vi "VIH Dialog - VI Terminals - Term Symbols.vi"(6 "cmd (nop)":T2(ring), 8 "error in":errorcluster, 11 "Ctl Refnum":refnum<vi>) -> (0 "error out":errorcluster, 1 "Symbols":T1[](array[typedef]), 2 "Symbol Index":i32, 3 "dup Ctl Refnum":refnum<vi>)   [LabVIEW 2014]
doc: "::: VI Helpeks :::\nCopyright (c) 2000-2026 Konstantin Shifershteyn. All rights reserved."
uses:
  <vilib>/picture/picture.llb/imagedata.ctl
panel:
  out "max Symbol Index":i32
  # "VI Helpeks\nCopyright (c) 2012-2026 Konstantin Shifershteyn"
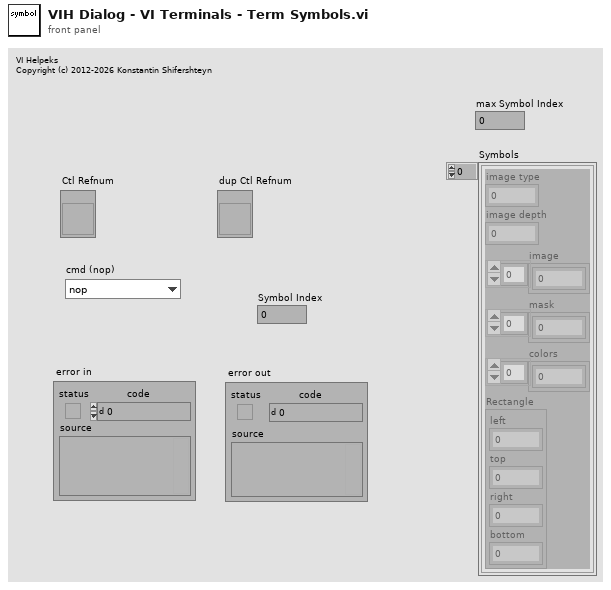
[diagram p1: front panel]
types:
  T1 = typedef "imagedata.ctl" = cluster{"image type":i32, "image depth":i32, "image":u8[], "mask":u8[], "colors":u32[], "Rectangle":cluster{"left":i16, "top":i16, "right":i16, "bottom":i16}}
  T2 = enum16{"nop", "Init", "get index", "get symbols"}
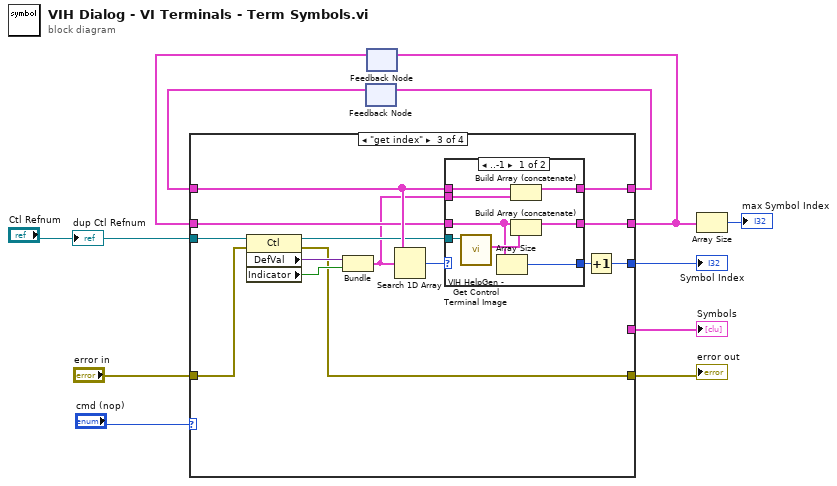
[diagram p0: block diagram]
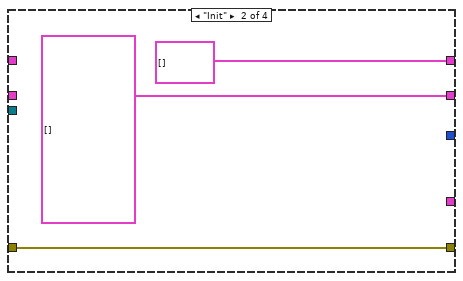
[diagram p3: hidden frame]
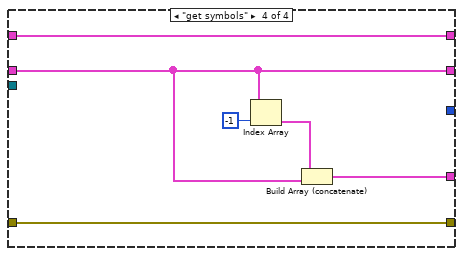
[diagram p5: hidden frame]
diagram:
  n1 = feedback #1() -> (w10:cluster{"DefVal":variant, "Indicator":bool}[])  [unwired: 1 in]
  n2 = feedback #2() -> (w9:T1[])  [unwired: 1 in]
  n3 = case shown="\"get index\"" "cmd (nop)" {
    tunnel: [w14 cluster{"DefVal":variant, "Indicator":bool}[] [] w31 w48] -> w11
    tunnel: w10 -> [w14 _ w30 w48]
    tunnel: w9 -> [w13 _ w29 w46]
    tunnel: [w13 T1[] [] w28 w46] -> w8
    tunnel: "Ctl Refnum" -> [_ _ w27 _]
    tunnel: [_ _ w18 _] -> w6
    tunnel: [_ _ _ w44] -> w4
    tunnel: "error in" -> [w12 w15 w20 w43]
    tunnel: [w12 w15 w19 w43] -> w2
    frame "nop" {
    }
    frame "Init" {
    }
    frame "get index" {
      n4 = property class="Ctl"(reference=w27, error in=w20) -> (reference out=w25:refnum<vi>, error out=w19:errorcluster, "DefVal"=w23:variant, "Indicator"=w22:bool)
      n5 = Bundle("DefVal"=w23, "Indicator"=w22) -> (w24:cluster{"DefVal":variant, "Indicator":bool})  [unwired: 1 in]
      n6 = Search 1D Array(1D array=w30, element=w24) -> (index of element=w26:i32)  [unwired: 1 in]
      n7 = case shown="..-1" w26 {
        selector: w26 -> [_ w41]
        tunnel: [w38 w42] -> w31
        tunnel: w30 -> [w39 w42]
        tunnel: w24 -> [w37 _]
        tunnel: [w34 w41] -> w21
        tunnel: [w33 w40] -> w28
        tunnel: w29 -> [w32 w40]
        tunnel: w25 -> [w36 _]
        frame ..-1 {
          n8 = call "VIH HelpGen - Get Control Terminal Image.vi"("Ctl Refnum"=w36) -> ("Ctrl Term Icon"=w35:T1)  [unwired: 6 in, 4 out]
          n9 = Array Size(array=w32) -> (size(s)=w34:i32)
          n10 = Build Array (concatenate)(w39, w37) -> (w38:cluster{"DefVal":variant, "Indicator":bool}[])
          n11 = Build Array (concatenate)(w32, w35) -> (w33:T1[])
        }
        frame 0.. {
        }
      }
      n12 = Increment(x=w21) -> (x+1=w18:i32)
    }
    frame "get symbols" {
      n13 = Index Array(array=w46, index=-1) -> (element=w45:T1)
      n14 = Build Array (concatenate)(w45, w46) -> (w44:T1[])
    }
  }
  "error out" <- w2
  "Symbol Index" <- w6
  "Symbols" <- w4
  n15 = feedback-in #1(w11) -> ()
  n16 = feedback-in #2(w8) -> ()
  n17 = Array Size(array=w8) -> (size(s)=→"max Symbol Index":i32)
  "dup Ctl Refnum" <- "Ctl Refnum"
